vi "HAL_Init.vi"() -> (0 "error out":errorcluster)   [LabVIEW 2023]
uses:
  wpiHal.so
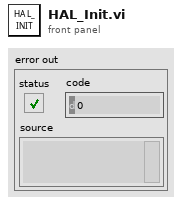
[diagram p1: front panel]
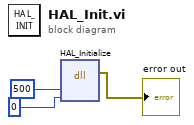
[diagram p0: block diagram]
diagram:
  n1 = dll-call lib="wpiHal.*" fn="HAL_Initialize"("arg1"=500, "arg2"=0) -> (error out=→"error out":errorcluster)  [unwired: 6 in, 1 out]
